vi "NSA Call Handover.vi"(8 "error in (no error)":errorcluster caption="에러 입력(에러 없음)", 10 "NSA Call Handover Param":T1, 11 "Instrument Manager 입력":refnum<class "Instrument Manager.lvclass">) -> (0 "error out":errorcluster caption="에러 출력", 3 "Instrument Manager 출력":refnum<class "Instrument Manager.lvclass">)   [LabVIEW 2023, in "Instrument Manager.lvclass"]
uses:
  Instrument Manager.lvclass
  Type Definition/NSA Call Handover Param.ctl
  Module/ANRITSU Call Box/Type Definition/NR Modulation Type.ctl
  c44f4119-fe54-4b2e-901b-91540a775e0b.vi
  Instrument Manager.lvclass/Instrument Manager.ctl
  eaf50d48-8f7c-4fb2-ae2e-7a07dcfe774a.vi
  Module/ANRITSU Call Box/ANRITSU Call Box.lvlib
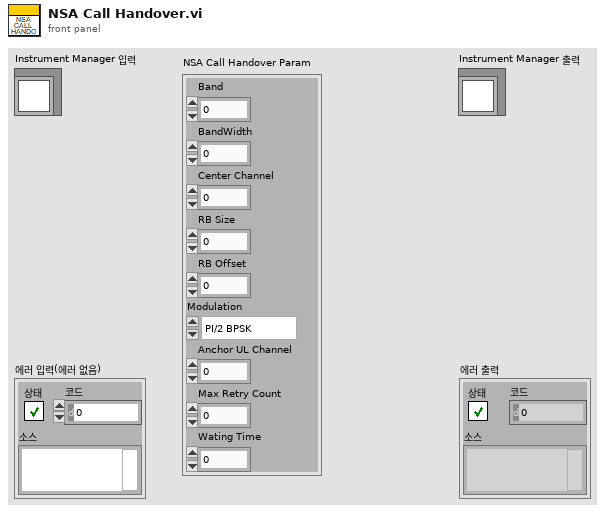
[diagram p1: front panel]
types:
  T1 = typedef "NSA Call Handover Param.ctl" = cluster{"Band":u32, "BandWidth":u32, "Center Channel":u32, "RB Size":i32, "RB Offset":i32, "Modulation":T2, "Anchor UL Channel":i32, "Max Retry Count":i32, "Wating Time":i32}
  T2 = typedef "ANRITSU Call Box.lvlib/NR Modulation Type.ctl" = enum16{"PI/2 BPSK", "QPSK", "16QAM", "64QAM", "256QAM"}
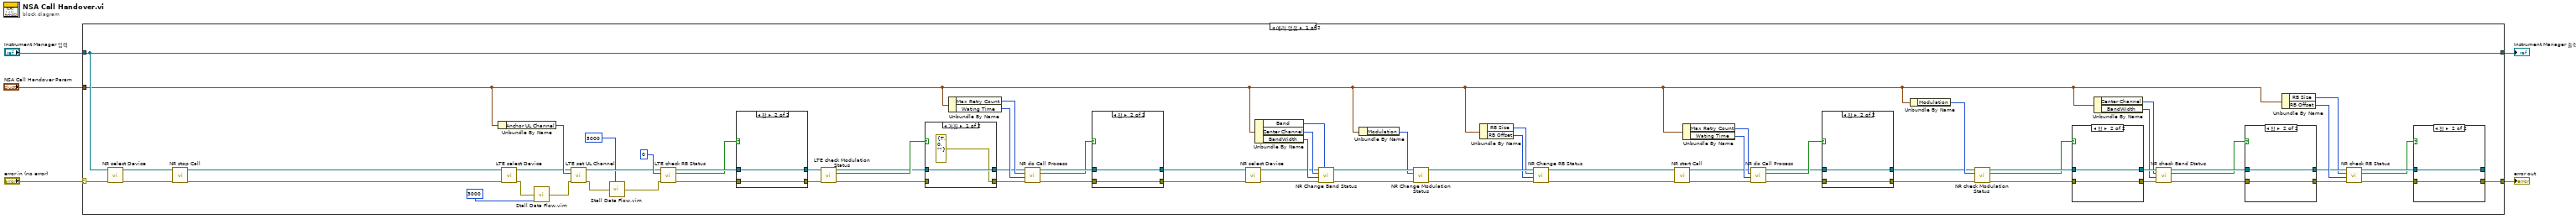
[diagram p0: block diagram]
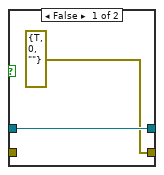
[diagram p2: hidden frame]
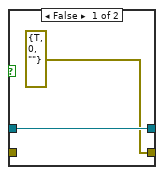
[diagram p4: hidden frame]
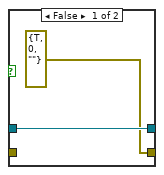
[diagram p5: hidden frame]
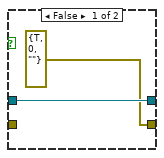
[diagram p6: hidden frame]
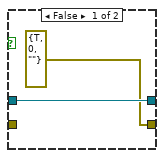
[diagram p7: hidden frame]
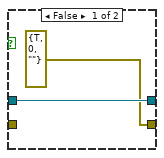
[diagram p8: hidden frame]
diagram:
  n1 = case shown="에러 없음" "error in (no error)" {
    selector: "error in (no error)" -> [w45 w111]
    tunnel: [w24 w111] -> w4
    tunnel: [w44 w110] -> w2
    tunnel: "Instrument Manager 입력" -> [w44 w110]
    tunnel: "NSA Call Handover Param" -> [w30 _]
    frame No Error {
      n2 = call "NR select Device.vi"("error in (no error)"=w45, "Instrument Manager 입력"=w44) -> ("error out"=w43:errorcluster, "Instrument Manager 출력"=w42:refnum<class "Instrument Manager.lvclass">)  [unwired: 8 in]
      n3 = call "NR stop Call.vi"("error in (no error)"=w43, "Instrument Manager 입력"=w42) -> ("error out"=w12:errorcluster, "Instrument Manager 출력"=w13:refnum<class "Instrument Manager.lvclass">)  [unwired: 8 in]
      n4 = Unbundle By Name(w30) -> ("Anchor UL Channel"=w81:i32)
      n5 = call "LTE select Device.vi"("error in (no error)"=w12, "Instrument Manager 입력"=w13) -> ("error out"=w8:errorcluster, "Instrument Manager 출력"=w39:refnum<class "Instrument Manager.lvclass">)  [unwired: 8 in]
      n6 = call "Stall Data Flow.vim"("value in"=w8, "milliseconds to wait"=u32 3000) -> ("value out"=w7:errorcluster)  [unwired: 1 out]
      n7 = call "LTE set UL Channel.vi"("error in (no error)"=w7, "UL Channel"=w81, "Instrument Manager 입력"=w39) -> ("error out"=w11:errorcluster, "Instrument Manager 출력"=w40:refnum<class "Instrument Manager.lvclass">)  [unwired: 7 in]
      n8 = call "Stall Data Flow.vim"("value in"=w11, "milliseconds to wait"=u32 5000) -> ("value out"=w10:errorcluster)  [unwired: 1 out]
      n9 = call "LTE check RB Status.vi"("error in (no error)"=w10, "RB Offset"=0, "Instrument Manager 입력"=w40) -> ("error out"=w38:errorcluster, "불리언"=w36:bool, "Instrument Manager 출력"=w37:refnum<class "Instrument Manager.lvclass">)  [unwired: 6 in]
      n10 = case shown="참" w36 {
        tunnel: w37 -> [w91 w93]
        tunnel: [w91 w93] -> w34
        tunnel: [errorcluster {"status"=TRUE, "code"=0, "source"=""} ("error out") w92] -> w35
        tunnel: w38 -> [_ w92]
        frame False {
        }
        frame True {
        }
      }
      n11 = call "LTE check Modulation Status.vi"("error in (no error)"=w35, "Instrument Manager 입력"=w34) -> ("error out"=w32:errorcluster, "불리언"=w33:bool, "Instrument Manager 출력"=w31:refnum<class "Instrument Manager.lvclass">)  [unwired: 7 in]
      n12 = case shown="거짓" w33 {
        tunnel: w31 -> [w87 w89]
        tunnel: [w87 w89] -> w19
        tunnel: [errorcluster {"status"=TRUE, "code"=0, "source"=""} ("error out") w88] -> w18
        tunnel: w32 -> [_ w88]
        frame False {
        }
        frame True {
        }
      }
      n13 = Unbundle By Name(w30) -> ("Max Retry Count"=w28:i32, "Wating Time"=w29:i32)
      n14 = call "NR do Call Process.vi"("error in (no error)"=w18, "Waiting Time"=w29, "Max Retry Count"=w28, "Instrument Manager 입력"=w19) -> ("error out"=w27:errorcluster, "Connected?"=w25:bool, "Instrument Manager 출력"=w26:refnum<class "Instrument Manager.lvclass">)  [unwired: 5 in]
      n15 = case shown="참" w25 {
        tunnel: w26 -> [w83 w85]
        tunnel: [w83 w85] -> w17
        tunnel: [errorcluster {"status"=TRUE, "code"=0, "source"=""} ("error out") w84] -> w16
        tunnel: w27 -> [_ w84]
        frame False {
        }
        frame True {
        }
      }
      n16 = call "NR select Device.vi"("error in (no error)"=w16, "Instrument Manager 입력"=w17) -> ("error out"=w15:errorcluster, "Instrument Manager 출력"=w14:refnum<class "Instrument Manager.lvclass">)  [unwired: 8 in]
      n17 = Unbundle By Name(w30) -> ("Band"=w66:u32, "Center Channel"=w67:u32, "BandWidth"=w68:u32)
      n18 = call "NR Change Band Status.vi"("Operation Band"=w66, "error in (no error)"=w15, "BW (MHz)"=w68, "Center Channel Number"=w67, "Instrument Manager 입력"=w14) -> ("error out"=w79:errorcluster, "Instrument Manager 출력"=w80:refnum<class "Instrument Manager.lvclass">)  [unwired: 5 in]
      n19 = Unbundle By Name(w30) -> ("Modulation"=w65:T2)
      n20 = call "NR Change Modulation Status.vi"("error in (no error)"=w79, "Modulation"=w65, "Instrument Manager 입력"=w80) -> ("error out"=w60:errorcluster, "Instrument Manager 출력"=w59:refnum<class "Instrument Manager.lvclass">)  [unwired: 7 in]
      n21 = Unbundle By Name(w30) -> ("RB Size"=w57:i32, "RB Offset"=w58:i32)
      n22 = call "NR Change RB Status.vi"("error in (no error)"=w60, "RB Offset"=w58, "RB Size"=w57, "Instrument Manager 입력"=w59) -> ("error out"=w23:errorcluster, "Instrument Manager 출력"=w21:refnum<class "Instrument Manager.lvclass">)  [unwired: 6 in]
      n23 = call "NR start Call.vi"("error in (no error)"=w23, "Instrument Manager 입력"=w21) -> ("error out"=w22:errorcluster, "Instrument Manager 출력"=w20:refnum<class "Instrument Manager.lvclass">)  [unwired: 8 in]
      n24 = Unbundle By Name(w30) -> ("Max Retry Count"=w49:i32, "Wating Time"=w50:i32)
      n25 = call "NR do Call Process.vi"("error in (no error)"=w22, "Waiting Time"=w50, "Max Retry Count"=w49, "Instrument Manager 입력"=w20) -> ("error out"=w51:errorcluster, "Connected?"=w53:bool, "Instrument Manager 출력"=w52:refnum<class "Instrument Manager.lvclass">)  [unwired: 5 in]
      n26 = case shown="참" w53 {
        tunnel: w52 -> [w95 w97]
        tunnel: [w95 w97] -> w47
        tunnel: [errorcluster {"status"=TRUE, "code"=0, "source"=""} ("error out") w96] -> w48
        tunnel: w51 -> [_ w96]
        frame False {
        }
        frame True {
        }
      }
      n27 = Unbundle By Name(w30) -> ("Modulation"=w64:T2)
      n28 = call "NR check Modulation Status.vi"("error in (no error)"=w48, "Modulation"=w64, "Instrument Manager 입력"=w47) -> ("error out"=w77:errorcluster, "Success?"=w72:bool, "Instrument Manager 출력"=w78:refnum<class "Instrument Manager.lvclass">)  [unwired: 6 in]
      n29 = case shown="참" w72 {
        tunnel: w78 -> [w107 w109]
        tunnel: [w107 w109] -> w76
        tunnel: [errorcluster {"status"=TRUE, "code"=0, "source"=""} ("error out") w108] -> w75
        tunnel: w77 -> [_ w108]
        frame False {
        }
        frame True {
        }
      }
      n30 = Unbundle By Name(w30) -> ("Center Channel"=w62:u32, "BandWidth"=w63:u32)
      n31 = call "NR check Band Status.vi"("error in (no error)"=w75, "BW (MHz)"=w63, "Center Channel Number"=w62, "Instrument Manager 입력"=w76) -> ("error out"=w74:errorcluster, "Success?"=w56:bool, "Instrument Manager 출력"=w73:refnum<class "Instrument Manager.lvclass">)  [unwired: 5 in]
      n32 = case shown="참" w56 {
        tunnel: w73 -> [w103 w105]
        tunnel: [w103 w105] -> w55
        tunnel: [errorcluster {"status"=TRUE, "code"=0, "source"=""} ("error out") w104] -> w54
        tunnel: w74 -> [_ w104]
        frame False {
        }
        frame True {
        }
      }
      n33 = Unbundle By Name(w30) -> ("RB Size"=w46:i32, "RB Offset"=w61:i32)
      n34 = call "NR check RB Status.vi"("error in (no error)"=w54, "RB Offset"=w61, "RB Size"=w46, "Instrument Manager 입력"=w55) -> ("error out"=w70:errorcluster, "Success?"=w69:bool, "Instrument Manager 출력"=w71:refnum<class "Instrument Manager.lvclass">)  [unwired: 5 in]
      n35 = case shown="참" w69 {
        tunnel: w71 -> [w99 w101]
        tunnel: [w99 w101] -> _
        tunnel: [errorcluster {"status"=TRUE, "code"=0, "source"=""} ("error out") w100] -> w24
        tunnel: w70 -> [_ w100]
        frame False {
        }
        frame True {
        }
      }
    }
    frame Error {
    }
  }
  "error out" <- w4
  "Instrument Manager 출력" <- w2
